vi "AWS_Sequence_Receipt.vi"(8 "error in":errorcluster caption="エラー入力", 9 "Save name":string, 11 "S array":T3(array[cluster])) -> (0 "error out":errorcluster caption="エラー出力", 2 "Base Array":string[][][](array[string]), 3 "SQ array":string[][](array[string]))   [LabVIEW 2018]
panel:
  out "DOWN":bool
  out "UP":bool
  in  "Function":bool
  in  "OK?":bool
  in  "index":i32
  out "ACond#":i32
  out "S New Info and MiN out":T1={"Sample Sequence"="GATGATGATGATGATGAT", "Right Read MIN"=6, "Filter P"=0, "STD Type"=enum."Region", "Base Table"=[], "Selection"=enum."10kHz", "noise MAX"=3, "Sample name"=""} {"Base Table"."Value 3" format="%.2g"}
  out "Array":string[](array[string])
  out "subarray":string[][](array[string])
  out "size(s)":i32
  out "element":i32
  out "Base Table":T2(array[cluster])
  out "path":path
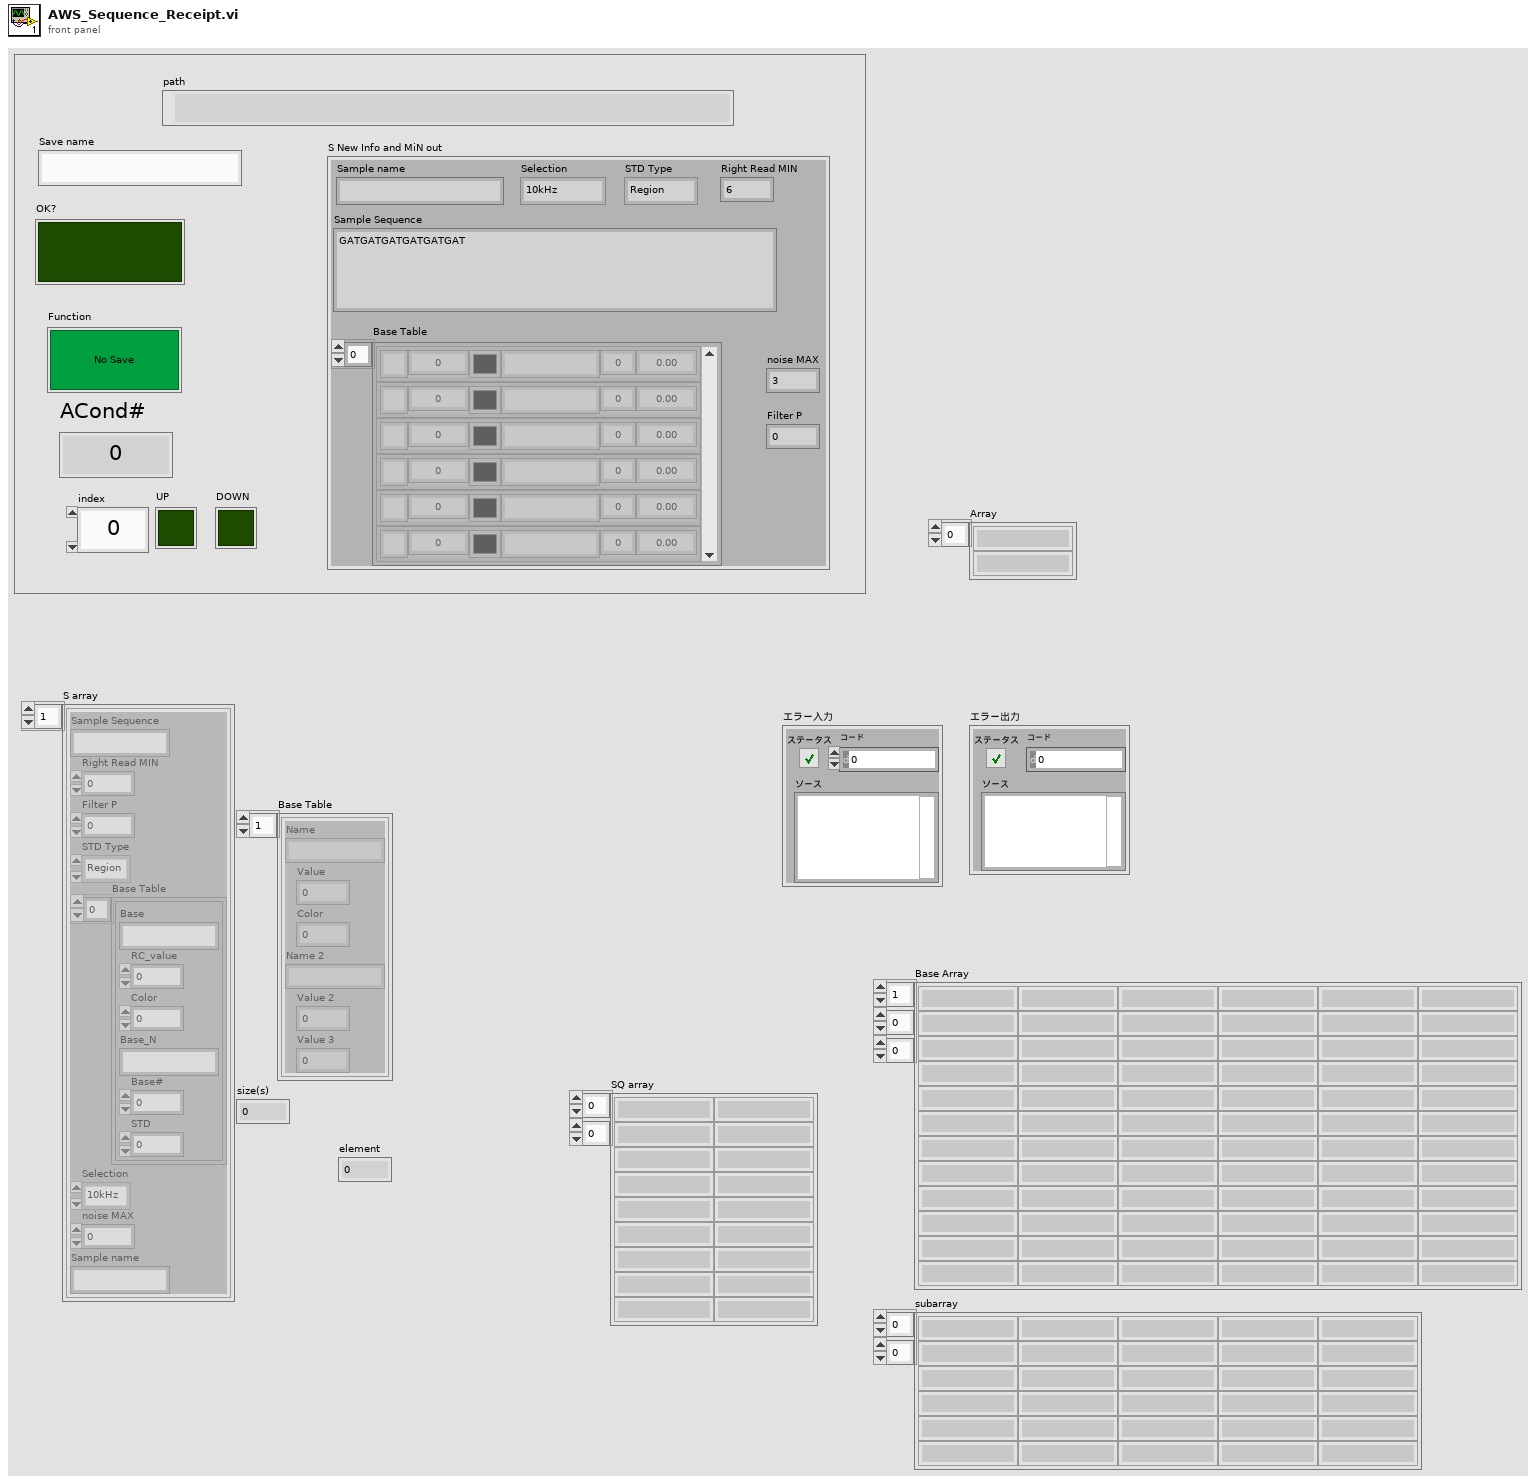
[diagram p1: front panel]
types:
  T1 = cluster{"Sample Sequence":string, "Right Read MIN":i32, "Filter P":i32, "STD Type":enum16{"Region", "Each", "Fixed"}, "Base Table":cluster{"Name":string, "Value":dbl, "Color":u32, "Name 2":string, "Value 2":dbl, "Value 3":dbl}[], "Selection":enum16{"10kHz", "100kHz"}, "noise MAX":i32, "Sample name":string}
  T2 = cluster{"Name":string, "Value":dbl, "Color":u32, "Name 2":string, "Value 2":dbl, "Value 3":dbl}[]
  T3 = cluster{"Sample Sequence":string, "Right Read MIN":i32, "Filter P":i32, "STD Type":enum16{"Region", "Each", "Fixed"}, "Base Table":cluster{"Base":string, "RC_value":dbl, "Color":u32, "Base_N":string, "Base#":dbl, "STD":dbl}[], "Selection":enum16{"10kHz", "100kHz"}, "noise MAX":i32, "Sample name":string}[]
  T4 = cluster{"Sample Sequence":string, "Right Read MIN":i32, "Filter P":i32, "STD Type":enum16{"Region", "Each", "Fixed"}, "Base Table":cluster{"Base":string, "RC_value":dbl, "Color":u32, "Base_N":string, "Base#":dbl, "STD":dbl}[], "Selection":enum16{"10kHz", "100kHz"}, "noise MAX":i32, "Sample name":string}
  T5 = enum16{"open", "open or create", "create or replace", "create", "open (read-only)"}
  T6 = cluster{"Base":string, "RC_value":dbl, "Color":u32, "Base_N":string, "Base#":dbl, "STD":dbl}[]
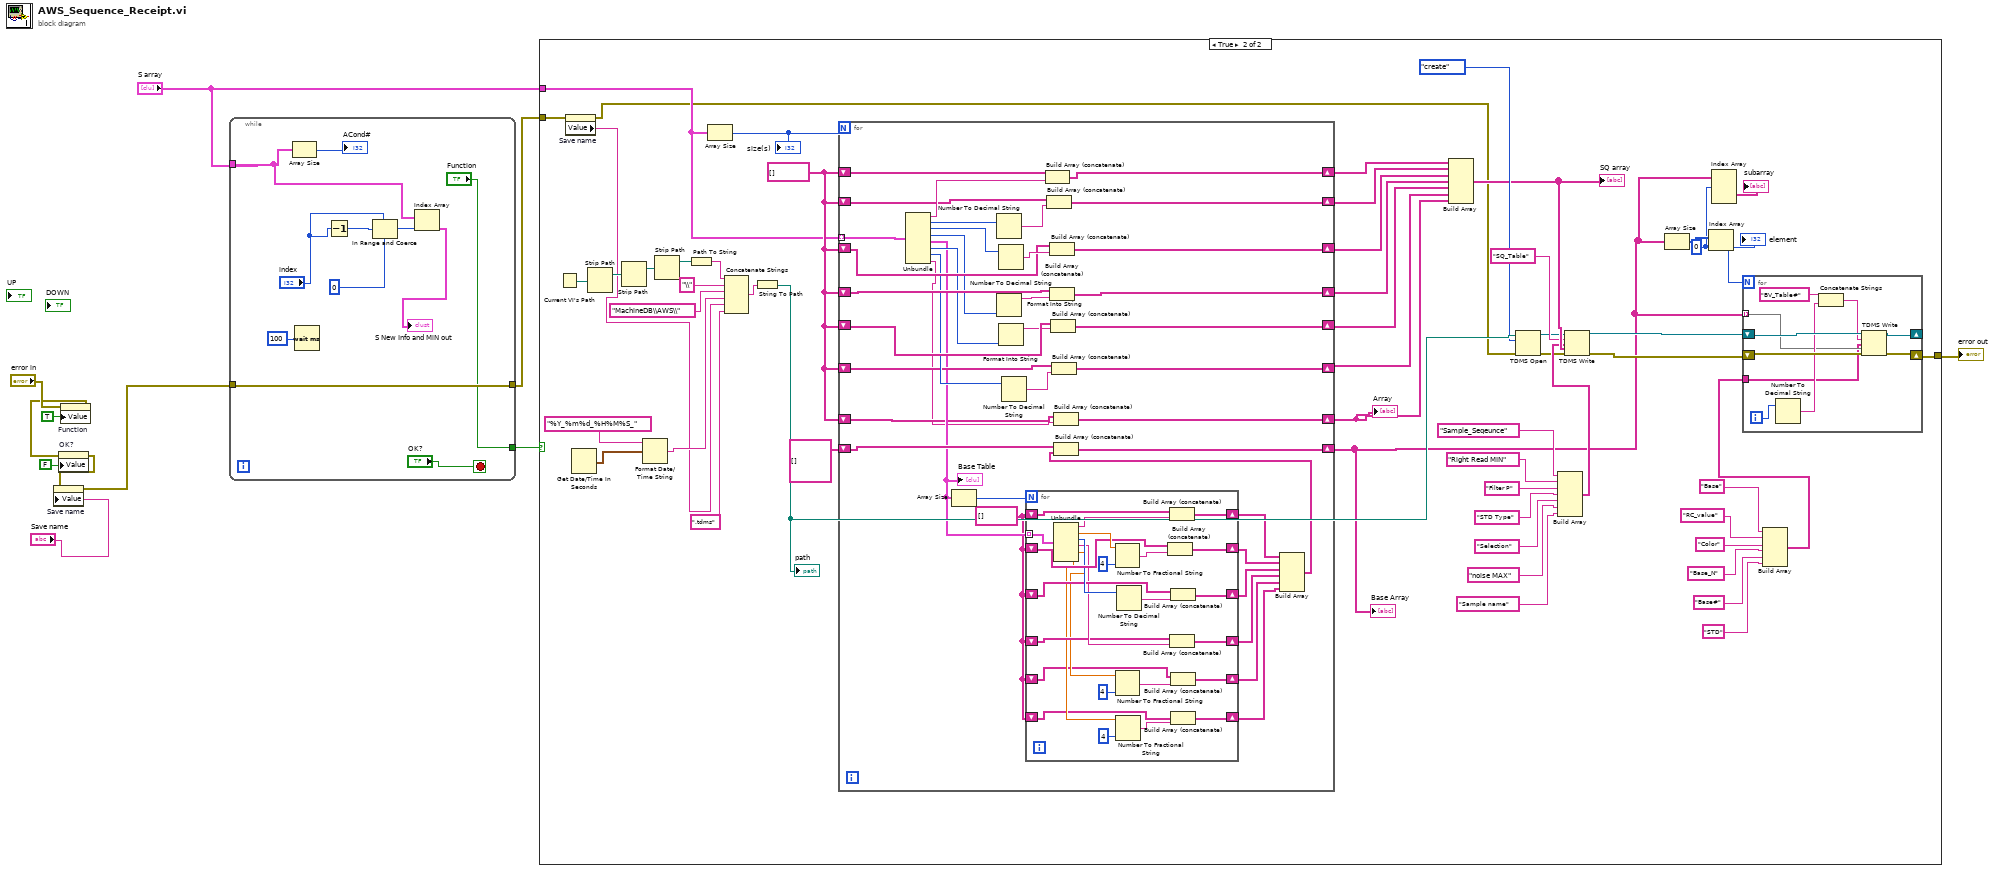
[diagram p0: block diagram]
diagram:
  n1 = property on="Function" class="Bool (strict)"(error in="error in", "Value"=TRUE ("Function")) -> (error out=w4:errorcluster)  [unwired: 1 in, 1 out]
  n2 = property on="OK?" class="Bool (strict)"(error in=w4, "Value"=FALSE ("OK?")) -> (error out=w2:errorcluster)  [unwired: 1 in, 1 out]
  n3 = property on="Save name" class="Str"(error in=w2, "Value"="Save name") -> (error out=w1:errorcluster)  [unwired: 1 in, 1 out]
  n4 = while {
    tunnel: w1 -> [w22]
    tunnel: [w22] -> w10
    tunnel: "S array" -> [w15]
    tunnel: ["Function"] -> w8
    stop <- "OK?" stop-if-true
    n5 = Array Size(array=w15) -> (size(s)=→"ACond#":i32)
    n6 = Wait (ms)(milliseconds to wait=u32 100) -> ()  [unwired: 1 out]
    n7 = Decrement(x="index") -> (x-1=w19:i32)
    n8 = In Range and Coerce(upper limit="index", x=w19, lower limit=0) -> (coerced(x)=w20:i32)  [unwired: 1 out]
    n9 = Index Array(array=w15, index=w20) -> (element=→"S New Info and MiN out":T4)
  }
  n10 = case shown="True" w8 {
    tunnel: [w23 w39] -> w11
    tunnel: w10 -> [w23 w26]
    tunnel: "S array" -> [_ w27]
    frame False {
    }
    frame True {
      w44 = 0 ("index")
      w64 = string[] []
      n11 = Current VI's Path() -> (path=w77:path)
      n12 = property on="Save name" class="Str"(error in=w26) -> (error out=w25:errorcluster, "Value"=w24:string)  [unwired: 1 in, 1 out]
      n13 = Get Date/Time In Seconds() -> (seconds since 1Jan1904=w29:timestamp)
      n14 = Strip Path(path=w77) -> (stripped path=w76:path)  [unwired: 1 out]
      n15 = Strip Path(path=w76) -> (stripped path=w75:path)  [unwired: 1 out]
      n16 = Format Date/Time String(time format string (%c)="%Y_%m%d_%H%M%S_" ("時間形式文字列（%c）"), seconds (now)=w29) -> (date/time string=w67:string)  [unwired: 1 in]
      n17 = Strip Path(path=w75) -> (stripped path=w74:path)  [unwired: 1 out]
      n18 = Path To String(path=w74) -> (string=w73:string)
      n19 = Array Size(array=w27) -> (size(s)=w78:i32)
      "size(s)" <- w78
      n20 = Concatenate Strings(w73, "\\" ("文字列"), "MachineDB\\AWS\\" ("文字列"), w67, w24, ".tdms" ("string")) -> (w70:string)
      n21 = String To Path(string=w70) -> (path=w66:path)
      "path" <- w66
      n22 = for {
        N: w78 -> [_]
        tunnel: w27 -> [w127] mode=indexing
        shift-right: [w125] -> w63
        shift-left: w64 -> [w124]
        shift-right: [w121] -> w62
        shift-left: w64 -> [w120]
        shift-right: [w119] -> w61
        shift-left: w64 -> [w116]
        shift-right: [w115] -> w60
        shift-left: w64 -> [w114]
        shift-right: [w113] -> w59
        shift-left: w64 -> [w112]
        shift-right: [w109] -> w58
        shift-left: w64 -> [w108]
        shift-right: [w107] -> w28
        shift-left: w64 -> [w90]
        shift-right: [w102] -> w37
        shift-left: string[][][] [] -> [w101]
        w98 = string[] []
        n23 = Unbundle(w127) -> ("Sample Sequence"=w126:string, "Right Read MIN"=w123:i32, "Filter P"=w118:i32, "STD Type"=w104:enum16{"Region", "Each", "Fixed"}, "Base Table"=w99:T6, "Selection"=w106:enum16{"10kHz", "100kHz"}, "noise MAX"=w111:i32, "Sample name"=w89:string)
        "Base Table" <- w99
        n24 = Array Size(array=w99) -> (size(s)=w100:i32)
        n25 = Number To Decimal String(number=w123) -> (decimal integer string=w122:string)  [unwired: 1 in]
        n26 = Format Into String(w104) -> (resulting string=w103:string)  [unwired: 3 in, 1 out]
        n27 = Number To Decimal String(number=w118) -> (decimal integer string=w117:string)  [unwired: 1 in]
        n28 = Format Into String(w106) -> (resulting string=w105:string)  [unwired: 3 in, 1 out]
        n29 = Number To Decimal String(number=w111) -> (decimal integer string=w110:string)  [unwired: 1 in]
        n30 = for {
          N: w100 -> [_]
          tunnel: w99 -> [w153] mode=indexing
          shift-right: [w151] -> w97
          shift-left: w98 -> [w150]
          shift-right: [w146] -> w96
          shift-left: w98 -> [w145]
          shift-right: [w142] -> w95
          shift-left: w98 -> [w141]
          shift-right: [w140] -> w94
          shift-left: w98 -> [w138]
          shift-right: [w132] -> w93
          shift-left: w98 -> [w131]
          shift-right: [w129] -> w92
          shift-left: w98 -> [w128]
          n31 = Unbundle(w153) -> ("Base"=w152:string, "RC_value"=w149:dbl, "Color"=w144:u32, "Base_N"=w139:string, "Base#"=w136:dbl, "STD"=w134:dbl)
          n32 = Number To Fractional String(number=w149, precision (6)=i16 4) -> (F-format string=w147:string)  [unwired: 2 in]
          n33 = Number To Fractional String(number=w136, precision (6)=i16 4) -> (F-format string=w133:string)  [unwired: 2 in]
          n34 = Number To Fractional String(number=w134, precision (6)=i16 4) -> (F-format string=w130:string)  [unwired: 2 in]
          n35 = Number To Decimal String(number=w144) -> (decimal integer string=w143:string)  [unwired: 1 in]
          n36 = Build Array (concatenate)(w145, w147) -> (w146:string[])
          n37 = Build Array (concatenate)(w150, w152) -> (w151:string[])
          n38 = Build Array (concatenate)(w138, w139) -> (w140:string[])
          n39 = Build Array (concatenate)(w141, w143) -> (w142:string[])
          n40 = Build Array (concatenate)(w131, w133) -> (w132:string[])
          n41 = Build Array (concatenate)(w128, w130) -> (w129:string[])
        }
        n42 = Build Array (concatenate)(w124, w126) -> (w125:string[])
        n43 = Build Array (concatenate)(w120, w122) -> (w121:string[])
        n44 = Build Array (concatenate)(w116, w117) -> (w119:string[])
        n45 = Build Array (concatenate)(w114, w103) -> (w115:string[])
        n46 = Build Array (concatenate)(w112, w105) -> (w113:string[])
        n47 = Build Array (concatenate)(w108, w110) -> (w109:string[])
        n48 = Build Array (concatenate)(w90, w89) -> (w107:string[])
        n49 = Build Array(w97, w96, w95, w94, w93, w92) -> (w91:string[][])
        n50 = Build Array (concatenate)(w101, w91) -> (w102:string[][][])
      }
      "Base Array" <- w37
      "Array" <- w28
      n51 = Build Array(w63, w62, w61, w60, w59, w58, w28) -> (w57:string[][])
      "SQ array" <- w57
      n52 = TDMS Open(8:w25, 10:T5."create" ("operation (0:open)"), 11:w66) -> (0:w41:errorcluster, 3:w42:refnum<k34>)  [unwired: 4 in]
      n53 = Build Array("Sample_Seqeunce" ("group name in (Untitled)"), "Right Read MIN" ("group name in (Untitled)"), "Filter P" ("group name in (Untitled)"), "STD Type" ("group name in (Untitled)"), "Selection" ("group name in (Untitled)"), "noise MAX" ("group name in (Untitled)"), "Sample name" ("group name in (Untitled)")) -> (w48:string[])
      n54 = TDMS Write(0:w42, 5:"SQ_Table" ("group name in (Untitled)"), 7:w48, 9:w57, 11:w41) -> (4:w38:refnum<k34>, 15:w40:errorcluster)  [unwired: 1 in, 2 out]
      n55 = Array Size(array=w37) -> (size(s)=w46:i32[])
      n56 = Index Array(array=w46, index=w44) -> (element=w45:i32)
      "element" <- w45
      n57 = Index Array(array=w37, index (dim 0)=w44) -> (element=→"subarray":string[][])  [unwired: 2 in]
      n58 = Build Array("Base" ("group name in (Untitled)"), "RC_value" ("group name in (Untitled)"), "Color" ("group name in (Untitled)"), "Base_N" ("group name in (Untitled)"), "Base#" ("group name in (Untitled)"), "STD" ("group name in (Untitled)")) -> (w30:string[])
      n59 = for {
        N: w45 -> [_]
        shift-right: [w87] -> w39
        shift-left: w40 -> [w88]
        shift-right: [w85] -> _
        shift-left: w38 -> [w86]
        tunnel: w37 -> [w81] mode=indexing
        tunnel: w30 -> [w80]
        i -> [w83]
        n60 = Number To Decimal String(number=w83) -> (decimal integer string=w82:string)  [unwired: 1 in]
        n61 = Concatenate Strings("BV_Table#" ("group name in (Untitled)"), w82) -> (w79:string)
        n62 = TDMS Write(0:w86, 5:w79, 7:w80, 9:w81, 11:w88) -> (4:w85:refnum<k34>, 15:w87:errorcluster)  [unwired: 1 in, 2 out]
      }
    }
  }
  "error out" <- w11
